vi "ZM-HWM-createResources.vi"(8 "error in (no error)":errorcluster, 11 "ZM-HWM-hardware_manager in":refnum<class "ZM-HWM-hardware_manager.lvclass">) -> (0 "error out":errorcluster, 3 "ZM-HWM-hardware_manager out":refnum<class "ZM-HWM-hardware_manager.lvclass">)   [LabVIEW 2020, in "ZM-HWM-hardware_manager.lvlib" / "ZM-HWM-hardware_manager.lvclass"]
doc: "Creates the hardware manager's resources in Pre Launch Init: the stop user event (ZM-HWM-createEvents). If that fails, it destroys what was created (ZM-HWM-close) and returns the original error, so the launch fails."
uses:
  ZM-HWM-hardware_manager.lvclass
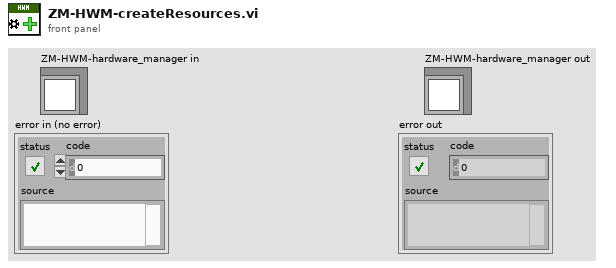
[diagram p1: front panel]
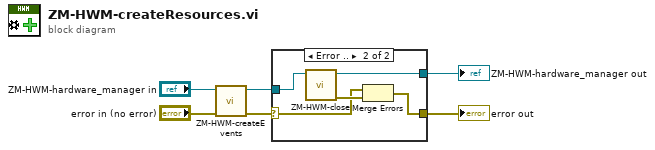
[diagram p0: block diagram]
diagram:
  n1 = call "ZM-HWM-createEvents.vi"("error in (no error)"="error in (no error)", "ZM-HWM-hardware_manager in"="ZM-HWM-hardware_manager in") -> ("error out"=w3:errorcluster, "ZM-HWM-hardware_manager out"=w4:refnum<class "ZM-HWM-hardware_manager.lvclass">)  [unwired: 8 in]
  n2 = case shown="Error .." w3 {
    selector: w3 -> [w7 w9]
    tunnel: w4 -> [w8 w13]
    tunnel: [w8 w11] -> w2
    tunnel: [w7 w10] -> w1
    frame No Error {
    }
    frame Error {
      n3 = call "ZM-HWM-close.vi"("ZM-HWM-hardware_manager in"=w13) -> ("error out"=w12:errorcluster, "ZM-HWM-hardware_manager out"=w11:refnum<class "ZM-HWM-hardware_manager.lvclass">)  [unwired: 9 in]
      n4 = Merge Errors(w9, w12) -> (w10:errorcluster)
    }
  }
  "ZM-HWM-hardware_manager out" <- w2
  "error out" <- w1
